vi "LabVIEW.HTTPs_Client.Test_Group.vi"(5 "Chose Server":string, 7 "Command":T1=enum."Test Label", 8 "Fehler (Eingang, kein Fehler)":errorcluster) -> (0 "Fehler (Ausgang)":errorcluster)   [LabVIEW 2026]
uses:
  LabVIEW.Type Definitions/LabVIEW.HTTPs_Client.Test_Group.Command.ctl
  LabVIEW.Type Definitions/LabVIEW.HTTPs_Client.Command.ctl
  <vilib>/JDP Science/JSONtext/String Subset.vi
  <vilib>/JDP Science/JSONtext/support/Strip Quotes and Unescape.vi
  <vilib>/JDP Science/JSONtext/support/Unescape JSON string.vi
  <vilib>/JDP Science/JSONtext/Parsing/Parse Full Path or Item Name.vi
  <vilib>/JDP Science/JSONtext/Offset/Find Item Locations by Path.vi
  <vilib>/JDP Science/JSONtext/JSONtext.lvlib
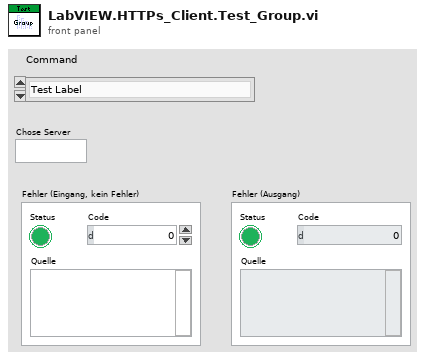
[diagram p1: front panel]
types:
  T1 = typedef "LabVIEW.HTTPs_Client.Test_Group.Command.ctl" = enum16{"No Command", " Test Authentication in the beginning", "Test Label", "Test Seriennummer", "Test Vorgang/Fertigung/Search", "Test User/Role/Permission", "Test MAC addresses", "Test Product/Product properties", "Test Health check", " Test Authentication at the end"}
  T2 = typedef "LabVIEW.HTTPs_Client.Command.ctl" = enum16{"Initialize HTTPS", "Authentication: Creat a token", "Authentication: Get all tokens", "Authentication: Revoke the token", "Label: Creat a label configuration", "Label: Get all configured labels", "Label: Update the label configuration", "Label: Delete the label configuration", "Label: Creat a colour ribbon", "Label: Update the colour ribbon", "Label: Get all colour ribbons", "Label: Delete the colour ribbon", "Label: Creat a label tape", "Label: Update the label tape", "Label: Get all label tapes", "Label: Delete the label tape", "Label: Get all label parameters", "Product: Get all product informations", "Product: Get all reading steps", "Seriennummer: Update the info text", "Seriennummer: Set all step states open", "Seriennummer: Update step states", "Seriennummer: Get data and steps", "Seriennummer: Get all label configurations", "Seriennummer: Create a text report(Prüfbericht)", "Seriennummer: Get the text report(Prüfbericht)", "Seriennummer: Delete the text report(Prüfbericht)", "Seriennummer: Upload a document(txt file)", "Seriennummer: Get the document", "Seriennummer: Get the document thumbnail", "Seriennummer: Delete the document", "Seriennummer: Bulk lookup", "Vorgang: Update the description text", "Vorgang: Migrate serial numbers to a Vorgang", "Vorgang: Migrate serial numbers to a product revision", "Vorgang: Update step states", "Vorgang: Create test reports(Prüfprotokoll)", "Vorgang: Get basic data", "Vorgang: Get serial number data and steps", "Vorgang: Get all serial numbers", "Vorgang: Generate a CSV file", "Vorgang: Generate an XLSX file", "Vorgang: Get a CSV file(Fertigmeldung report)", "Fertigmeldung: Create a Fertigmeldung", "Fertigmeldung: Revert the Fertigmeldung", "User: Get all users", "User: Update an user", "User: Get a single user", "User: Get all user roles", "User: Update a user role", "User: Get a single user role", "User: Get all permissions", "Search: Get Vorgang/Produkt combinations", "Search: Get Vorgang/Produkt/SN combinations", "Search: Get Seriennummern by Vorgang and Produkt", "Search: Lookup Vorgang", "MAC addresses: Get all reserved MAC addresses", "MAC addresses: Get the most recently reserved MAC addresses", "MAC addresses: Get data for a MAC address", "MAC addresses: Reserve MAC addresses for a Seriennummer", "MAC addresses: Mark a reserved MAC address as flashed", "Product: Get possible steps", "Product: Get all products", "Product: Create a new product", "Product: Update a product's data", "Product: Get next product IDs", "Product: Delete a product", "Product properties: Get all product property types", "Search: Find production plan", "Search: Find production plan arrangement", "Health check: Health check", "Deinitialize HTTPs"}
  T3 = enum16{"read csv", "clear csv", "read xlsx", "clear xlsx"}
  T4 = cluster{"Name":string, "URL":string, "Request body":string, "-H":string, "Hearder":string, "Bpdy":string}
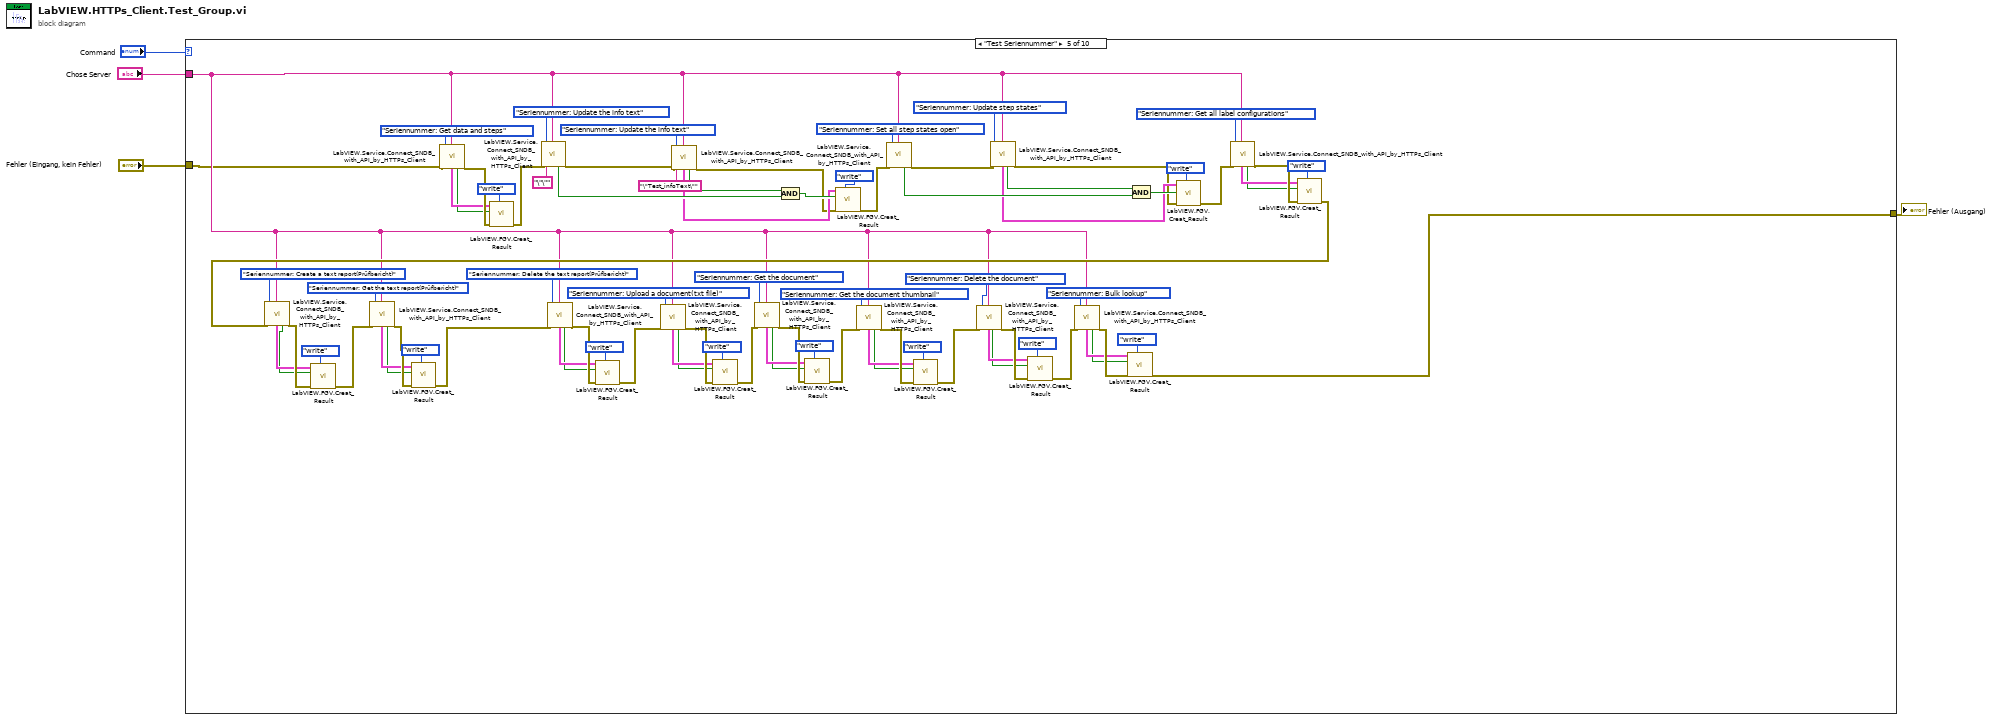
[diagram p0: block diagram]
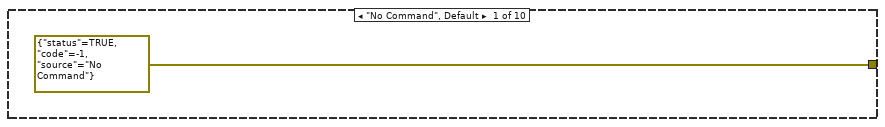
[diagram p2: hidden frame]
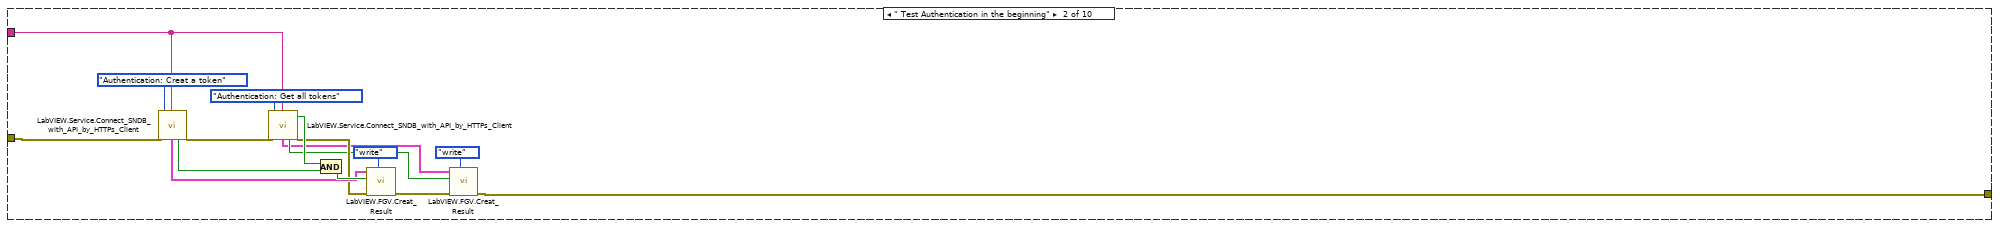
[diagram p3: hidden frame]
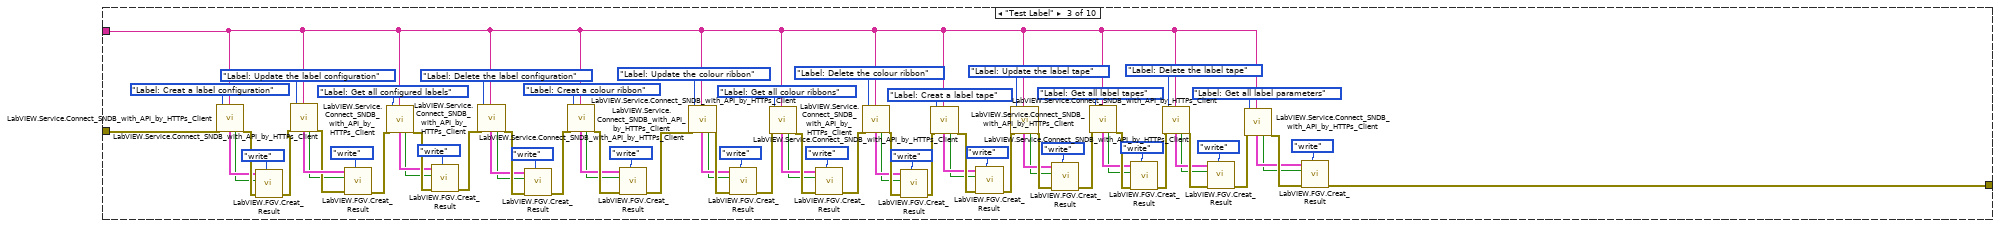
[diagram p4: hidden frame]
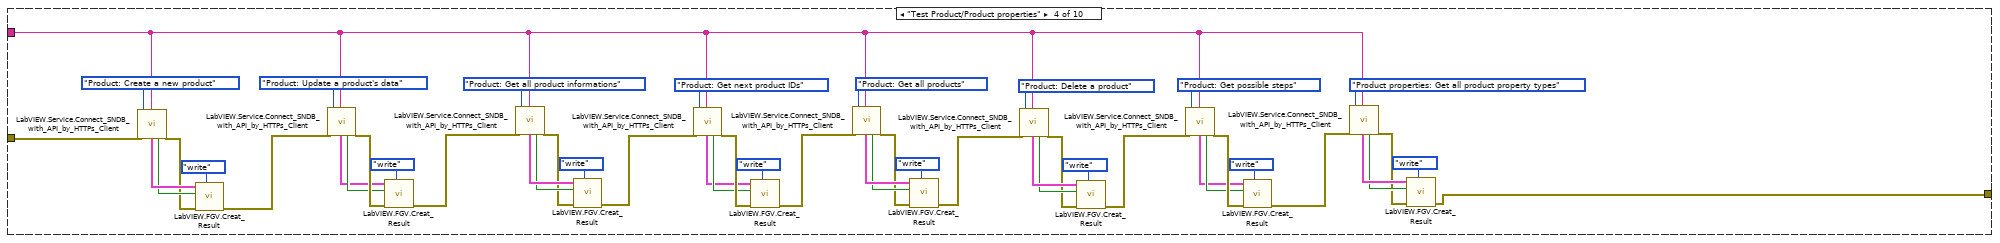
[diagram p5: hidden frame]
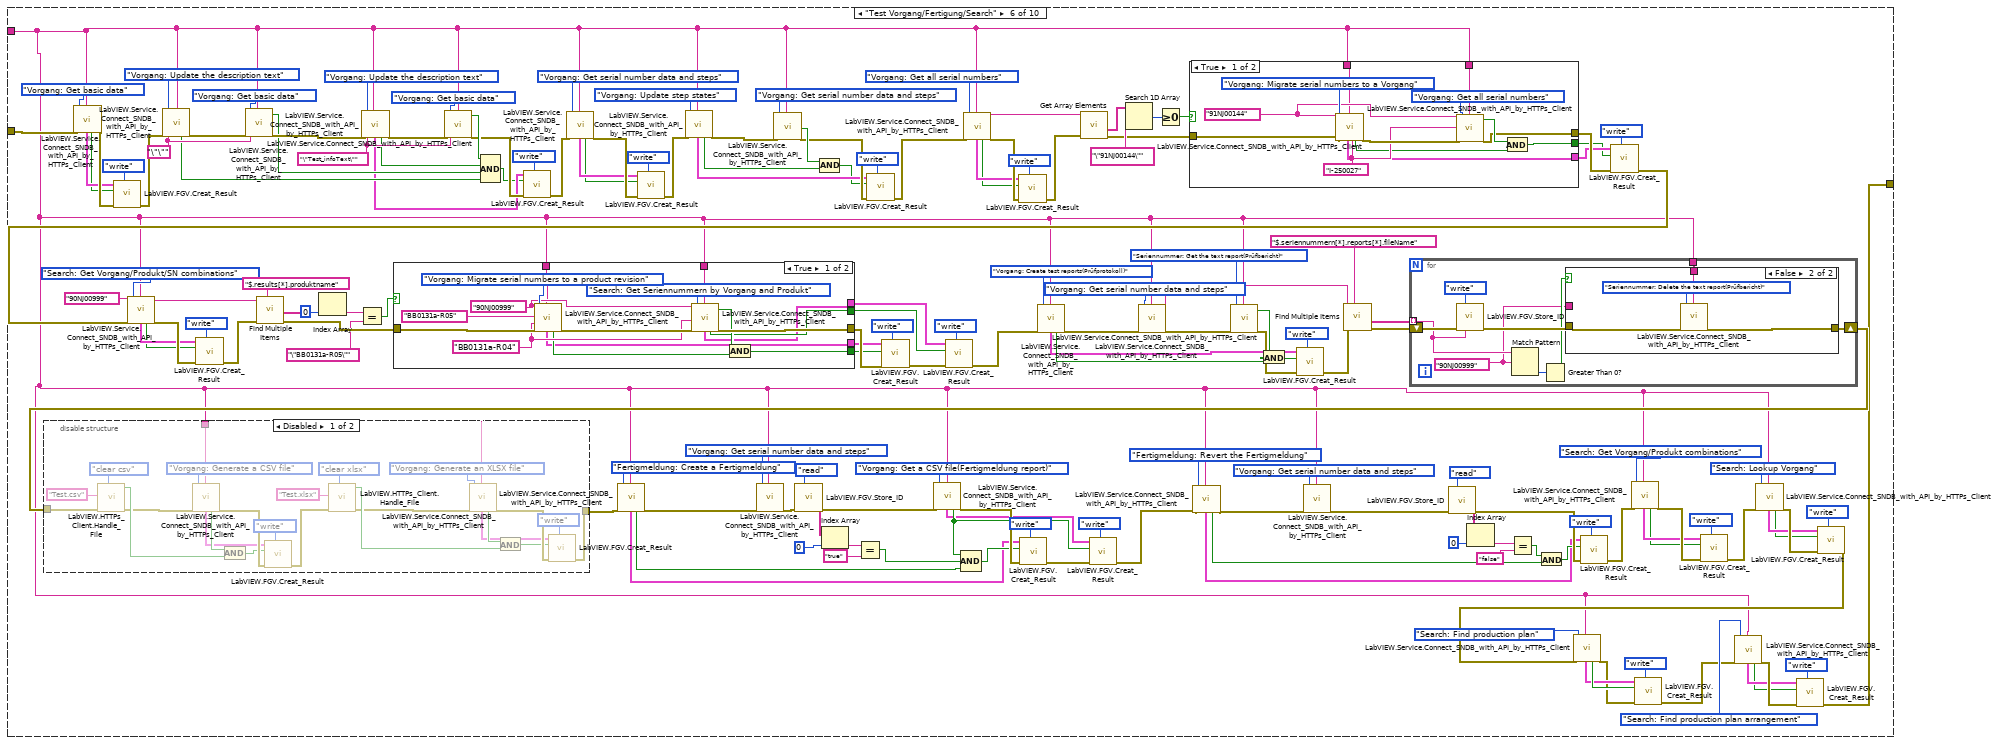
[diagram p6: hidden frame]
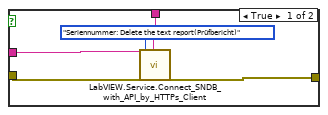
[diagram p8: hidden frame]
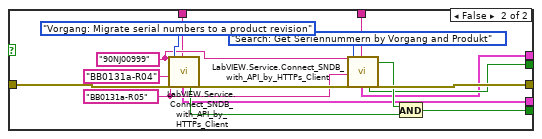
[diagram p9: hidden frame]
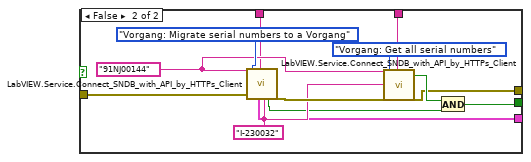
[diagram p10: hidden frame]
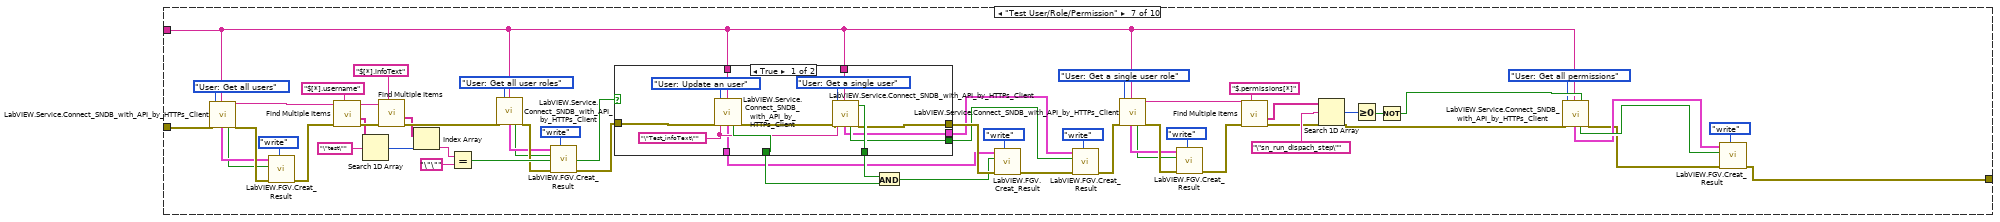
[diagram p11: hidden frame]
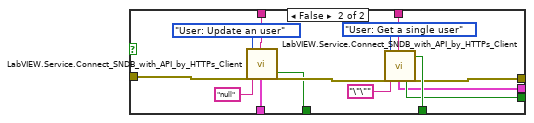
[diagram p12: hidden frame]
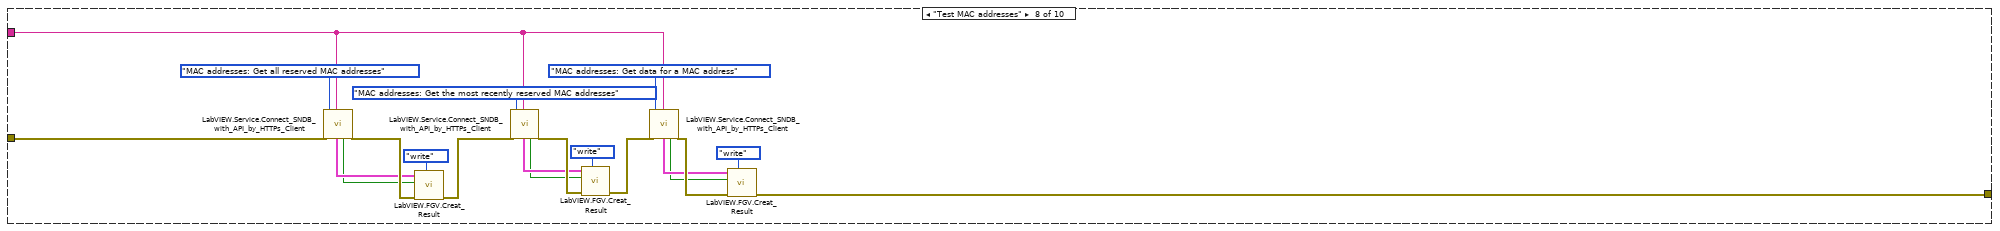
[diagram p13: hidden frame]
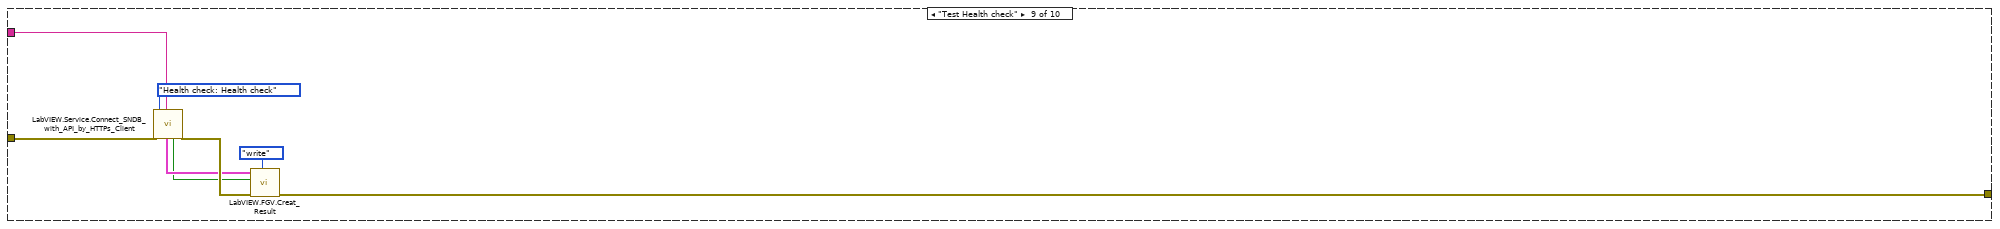
[diagram p14: hidden frame]
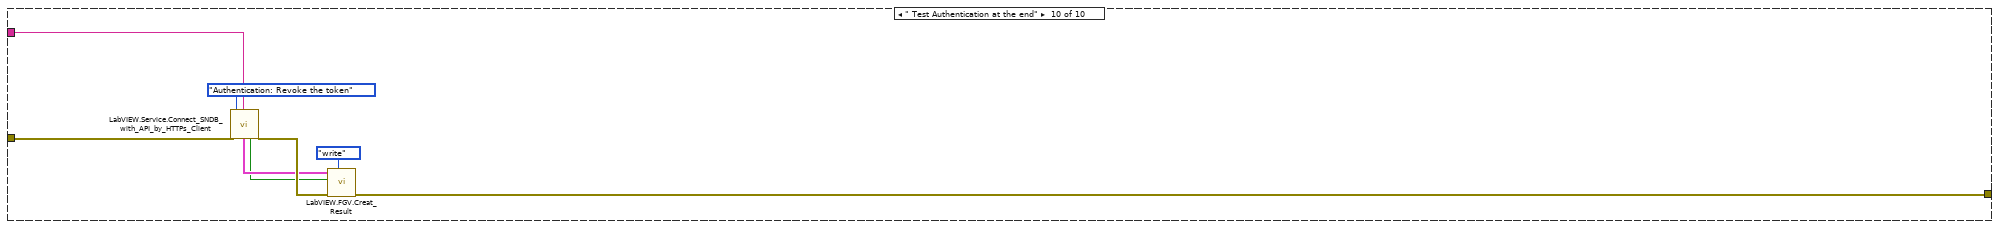
[diagram p15: hidden frame]
diagram:
  n1 = case shown="\"Test Seriennummer\"" "Command" {
    tunnel: "Fehler (Eingang, kein Fehler)" -> [_ w16 w101 w148 w154 w371 w531 w600 w605 w617]
    tunnel: [errorcluster {"status"=TRUE, "code"=-1, "source"="No Command"} ("error out") w7 w25 w102 w156 w237 w503 w587 w604 w615] -> w3
    tunnel: "Chose Server" -> [_ w6 w22 w103 w155 w236 w502 w584 w606 w612]
    frame "No Command", Default {
    }
    frame " Test Authentication in the beginning" {
      n2 = call "LabVIEW.Service.Connect_SNDB_with_API_by_HTTPs_Client.vi"("error in (no error)"=w16, "Command"=LabVIEW.HTTPs_Client.Command."Authentication: Creat a token", "Chose Server"=w6) -> ("Result_Cluster"=w13:T4, "Successful?"=w21:bool, "error out"=w17:errorcluster)  [unwired: 14 in, 8 out]
      n3 = call "LabVIEW.Service.Connect_SNDB_with_API_by_HTTPs_Client.vi"("error in (no error)"=w17, "Command"=LabVIEW.HTTPs_Client.Command."Authentication: Get all tokens", "Chose Server"=w6) -> ("Result_Cluster"=w8:T4, "Successful?"=w9:bool, "Test other steps"=w20:bool, "error out"=w12:errorcluster)  [unwired: 14 in, 7 out]
      n4 = And(x=w20, y=w21) -> (x .and. y?=w14:bool)
      n5 = call "LabVIEW.FGV.Creat_Result.vi"("Command"=enum16{"write", "read", "clear"}."write", "error in (no error)"=w12, "Passed?"=w14, "Result_Cluster"=w13) -> ("error out"=w10:errorcluster)  [unwired: 6 in, 1 out]
      n6 = call "LabVIEW.FGV.Creat_Result.vi"("Command"=enum16{"write", "read", "clear"}."write", "error in (no error)"=w10, "Passed?"=w9, "Result_Cluster"=w8) -> ("error out"=w7:errorcluster)  [unwired: 6 in, 1 out]
    }
    frame "Test Label" {
      n7 = call "LabVIEW.Service.Connect_SNDB_with_API_by_HTTPs_Client.vi"("error in (no error)"=w101, "Command"=LabVIEW.HTTPs_Client.Command."Label: Creat a label configuration", "Chose Server"=w22) -> ("Result_Cluster"=w84:T4, "Successful?"=w83:bool, "error out"=w87:errorcluster)  [unwired: 14 in, 8 out]
      n8 = call "LabVIEW.FGV.Creat_Result.vi"("Command"=enum16{"write", "read", "clear"}."write", "error in (no error)"=w87, "Passed?"=w83, "Result_Cluster"=w84) -> ("error out"=w86:errorcluster)  [unwired: 6 in, 1 out]
      n9 = call "LabVIEW.Service.Connect_SNDB_with_API_by_HTTPs_Client.vi"("error in (no error)"=w86, "Command"=LabVIEW.HTTPs_Client.Command."Label: Update the label configuration", "Chose Server"=w22) -> ("Result_Cluster"=w81:T4, "Successful?"=w78:bool, "error out"=w80:errorcluster)  [unwired: 14 in, 8 out]
      n10 = call "LabVIEW.FGV.Creat_Result.vi"("Command"=enum16{"write", "read", "clear"}."write", "error in (no error)"=w80, "Passed?"=w78, "Result_Cluster"=w81) -> ("error out"=w79:errorcluster)  [unwired: 6 in, 1 out]
      n11 = call "LabVIEW.Service.Connect_SNDB_with_API_by_HTTPs_Client.vi"("error in (no error)"=w79, "Command"=LabVIEW.HTTPs_Client.Command."Label: Get all configured labels", "Chose Server"=w22) -> ("Result_Cluster"=w74:T4, "Successful?"=w73:bool, "error out"=w76:errorcluster)  [unwired: 14 in, 8 out]
      n12 = call "LabVIEW.FGV.Creat_Result.vi"("Command"=enum16{"write", "read", "clear"}."write", "error in (no error)"=w76, "Passed?"=w73, "Result_Cluster"=w74) -> ("error out"=w75:errorcluster)  [unwired: 6 in, 1 out]
      n13 = call "LabVIEW.Service.Connect_SNDB_with_API_by_HTTPs_Client.vi"("error in (no error)"=w75, "Command"=LabVIEW.HTTPs_Client.Command."Label: Delete the label configuration", "Chose Server"=w22) -> ("Result_Cluster"=w69:T4, "Successful?"=w68:bool, "error out"=w71:errorcluster)  [unwired: 14 in, 8 out]
      n14 = call "LabVIEW.FGV.Creat_Result.vi"("Command"=enum16{"write", "read", "clear"}."write", "error in (no error)"=w71, "Passed?"=w68, "Result_Cluster"=w69) -> ("error out"=w70:errorcluster)  [unwired: 6 in, 1 out]
      n15 = call "LabVIEW.Service.Connect_SNDB_with_API_by_HTTPs_Client.vi"("error in (no error)"=w70, "Command"=LabVIEW.HTTPs_Client.Command."Label: Creat a colour ribbon", "Chose Server"=w22) -> ("Result_Cluster"=w64:T4, "Successful?"=w63:bool, "error out"=w66:errorcluster)  [unwired: 14 in, 8 out]
      n16 = call "LabVIEW.FGV.Creat_Result.vi"("Command"=enum16{"write", "read", "clear"}."write", "error in (no error)"=w66, "Passed?"=w63, "Result_Cluster"=w64) -> ("error out"=w65:errorcluster)  [unwired: 6 in, 1 out]
      n17 = call "LabVIEW.Service.Connect_SNDB_with_API_by_HTTPs_Client.vi"("error in (no error)"=w65, "Command"=LabVIEW.HTTPs_Client.Command."Label: Update the colour ribbon", "Chose Server"=w22) -> ("Result_Cluster"=w60:T4, "Successful?"=w59:bool, "error out"=w61:errorcluster)  [unwired: 14 in, 8 out]
      n18 = call "LabVIEW.FGV.Creat_Result.vi"("Command"=enum16{"write", "read", "clear"}."write", "error in (no error)"=w61, "Passed?"=w59, "Result_Cluster"=w60) -> ("error out"=w58:errorcluster)  [unwired: 6 in, 1 out]
      n19 = call "LabVIEW.Service.Connect_SNDB_with_API_by_HTTPs_Client.vi"("error in (no error)"=w58, "Command"=LabVIEW.HTTPs_Client.Command."Label: Get all colour ribbons", "Chose Server"=w22) -> ("Result_Cluster"=w54:T4, "Successful?"=w53:bool, "error out"=w56:errorcluster)  [unwired: 14 in, 8 out]
      n20 = call "LabVIEW.FGV.Creat_Result.vi"("Command"=enum16{"write", "read", "clear"}."write", "error in (no error)"=w56, "Passed?"=w53, "Result_Cluster"=w54) -> ("error out"=w55:errorcluster)  [unwired: 6 in, 1 out]
      n21 = call "LabVIEW.Service.Connect_SNDB_with_API_by_HTTPs_Client.vi"("error in (no error)"=w55, "Command"=LabVIEW.HTTPs_Client.Command."Label: Delete the colour ribbon", "Chose Server"=w22) -> ("Result_Cluster"=w49:T4, "Successful?"=w48:bool, "error out"=w51:errorcluster)  [unwired: 14 in, 8 out]
      n22 = call "LabVIEW.FGV.Creat_Result.vi"("Command"=enum16{"write", "read", "clear"}."write", "error in (no error)"=w51, "Passed?"=w48, "Result_Cluster"=w49) -> ("error out"=w50:errorcluster)  [unwired: 6 in, 1 out]
      n23 = call "LabVIEW.Service.Connect_SNDB_with_API_by_HTTPs_Client.vi"("error in (no error)"=w50, "Command"=LabVIEW.HTTPs_Client.Command."Label: Creat a label tape", "Chose Server"=w22) -> ("Result_Cluster"=w44:T4, "Successful?"=w43:bool, "error out"=w46:errorcluster)  [unwired: 14 in, 8 out]
      n24 = call "LabVIEW.FGV.Creat_Result.vi"("Command"=enum16{"write", "read", "clear"}."write", "error in (no error)"=w46, "Passed?"=w43, "Result_Cluster"=w44) -> ("error out"=w45:errorcluster)  [unwired: 6 in, 1 out]
      n25 = call "LabVIEW.Service.Connect_SNDB_with_API_by_HTTPs_Client.vi"("error in (no error)"=w45, "Command"=LabVIEW.HTTPs_Client.Command."Label: Update the label tape", "Chose Server"=w22) -> ("Result_Cluster"=w39:T4, "Successful?"=w38:bool, "error out"=w41:errorcluster)  [unwired: 14 in, 8 out]
      n26 = call "LabVIEW.FGV.Creat_Result.vi"("Command"=enum16{"write", "read", "clear"}."write", "error in (no error)"=w41, "Passed?"=w38, "Result_Cluster"=w39) -> ("error out"=w40:errorcluster)  [unwired: 6 in, 1 out]
      n27 = call "LabVIEW.Service.Connect_SNDB_with_API_by_HTTPs_Client.vi"("error in (no error)"=w40, "Command"=LabVIEW.HTTPs_Client.Command."Label: Get all label tapes", "Chose Server"=w22) -> ("Result_Cluster"=w34:T4, "Successful?"=w33:bool, "error out"=w36:errorcluster)  [unwired: 14 in, 8 out]
      n28 = call "LabVIEW.FGV.Creat_Result.vi"("Command"=enum16{"write", "read", "clear"}."write", "error in (no error)"=w36, "Passed?"=w33, "Result_Cluster"=w34) -> ("error out"=w35:errorcluster)  [unwired: 6 in, 1 out]
      n29 = call "LabVIEW.Service.Connect_SNDB_with_API_by_HTTPs_Client.vi"("error in (no error)"=w35, "Command"=LabVIEW.HTTPs_Client.Command."Label: Delete the label tape", "Chose Server"=w22) -> ("Result_Cluster"=w30:T4, "Successful?"=w29:bool, "error out"=w31:errorcluster)  [unwired: 14 in, 8 out]
      n30 = call "LabVIEW.FGV.Creat_Result.vi"("Command"=enum16{"write", "read", "clear"}."write", "error in (no error)"=w31, "Passed?"=w29, "Result_Cluster"=w30) -> ("error out"=w28:errorcluster)  [unwired: 6 in, 1 out]
      n31 = call "LabVIEW.Service.Connect_SNDB_with_API_by_HTTPs_Client.vi"("error in (no error)"=w28, "Command"=LabVIEW.HTTPs_Client.Command."Label: Get all label parameters", "Chose Server"=w22) -> ("Result_Cluster"=w24:T4, "Successful?"=w23:bool, "error out"=w26:errorcluster)  [unwired: 14 in, 8 out]
      n32 = call "LabVIEW.FGV.Creat_Result.vi"("Command"=enum16{"write", "read", "clear"}."write", "error in (no error)"=w26, "Passed?"=w23, "Result_Cluster"=w24) -> ("error out"=w25:errorcluster)  [unwired: 6 in, 1 out]
    }
    frame "Test Product/Product properties" {
      n33 = call "LabVIEW.Service.Connect_SNDB_with_API_by_HTTPs_Client.vi"("error in (no error)"=w148, "Command"=LabVIEW.HTTPs_Client.Command."Product: Create a new product", "Chose Server"=w103) -> ("Result_Cluster"=w150:T4, "Successful?"=w149:bool, "error out"=w146:errorcluster)  [unwired: 14 in, 8 out]
      n34 = call "LabVIEW.FGV.Creat_Result.vi"("Command"=enum16{"write", "read", "clear"}."write", "error in (no error)"=w146, "Passed?"=w149, "Result_Cluster"=w150) -> ("error out"=w140:errorcluster)  [unwired: 6 in, 1 out]
      n35 = call "LabVIEW.Service.Connect_SNDB_with_API_by_HTTPs_Client.vi"("error in (no error)"=w140, "Command"=LabVIEW.HTTPs_Client.Command."Product: Update a product's data", "Chose Server"=w103) -> ("Result_Cluster"=w142:T4, "Successful?"=w143:bool, "error out"=w145:errorcluster)  [unwired: 14 in, 8 out]
      n36 = call "LabVIEW.FGV.Creat_Result.vi"("Command"=enum16{"write", "read", "clear"}."write", "error in (no error)"=w145, "Passed?"=w143, "Result_Cluster"=w142) -> ("error out"=w134:errorcluster)  [unwired: 6 in, 1 out]
      n37 = call "LabVIEW.Service.Connect_SNDB_with_API_by_HTTPs_Client.vi"("error in (no error)"=w134, "Command"=LabVIEW.HTTPs_Client.Command."Product: Get all product informations", "Chose Server"=w103) -> ("Result_Cluster"=w138:T4, "Successful?"=w137:bool, "error out"=w135:errorcluster)  [unwired: 14 in, 8 out]
      n38 = call "LabVIEW.FGV.Creat_Result.vi"("Command"=enum16{"write", "read", "clear"}."write", "error in (no error)"=w135, "Passed?"=w137, "Result_Cluster"=w138) -> ("error out"=w128:errorcluster)  [unwired: 6 in, 1 out]
      n39 = call "LabVIEW.Service.Connect_SNDB_with_API_by_HTTPs_Client.vi"("error in (no error)"=w128, "Command"=LabVIEW.HTTPs_Client.Command."Product: Get next product IDs", "Chose Server"=w103) -> ("Result_Cluster"=w130:T4, "Successful?"=w131:bool, "error out"=w133:errorcluster)  [unwired: 14 in, 8 out]
      n40 = call "LabVIEW.FGV.Creat_Result.vi"("Command"=enum16{"write", "read", "clear"}."write", "error in (no error)"=w133, "Passed?"=w131, "Result_Cluster"=w130) -> ("error out"=w122:errorcluster)  [unwired: 6 in, 1 out]
      n41 = call "LabVIEW.Service.Connect_SNDB_with_API_by_HTTPs_Client.vi"("error in (no error)"=w122, "Command"=LabVIEW.HTTPs_Client.Command."Product: Get all products", "Chose Server"=w103) -> ("Result_Cluster"=w126:T4, "Successful?"=w125:bool, "error out"=w123:errorcluster)  [unwired: 14 in, 8 out]
      n42 = call "LabVIEW.FGV.Creat_Result.vi"("Command"=enum16{"write", "read", "clear"}."write", "error in (no error)"=w123, "Passed?"=w125, "Result_Cluster"=w126) -> ("error out"=w111:errorcluster)  [unwired: 6 in, 1 out]
      n43 = call "LabVIEW.Service.Connect_SNDB_with_API_by_HTTPs_Client.vi"("error in (no error)"=w111, "Command"=LabVIEW.HTTPs_Client.Command."Product: Delete a product", "Chose Server"=w103) -> ("Result_Cluster"=w115:T4, "Successful?"=w114:bool, "error out"=w112:errorcluster)  [unwired: 14 in, 8 out]
      n44 = call "LabVIEW.FGV.Creat_Result.vi"("Command"=enum16{"write", "read", "clear"}."write", "error in (no error)"=w112, "Passed?"=w114, "Result_Cluster"=w115) -> ("error out"=w105:errorcluster)  [unwired: 6 in, 1 out]
      n45 = call "LabVIEW.Service.Connect_SNDB_with_API_by_HTTPs_Client.vi"("error in (no error)"=w105, "Command"=LabVIEW.HTTPs_Client.Command."Product: Get possible steps", "Chose Server"=w103) -> ("Result_Cluster"=w118:T4, "Successful?"=w119:bool, "error out"=w121:errorcluster)  [unwired: 14 in, 8 out]
      n46 = call "LabVIEW.FGV.Creat_Result.vi"("Command"=enum16{"write", "read", "clear"}."write", "error in (no error)"=w121, "Passed?"=w119, "Result_Cluster"=w118) -> ("error out"=w104:errorcluster)  [unwired: 6 in, 1 out]
      n47 = call "LabVIEW.Service.Connect_SNDB_with_API_by_HTTPs_Client.vi"("error in (no error)"=w104, "Command"=LabVIEW.HTTPs_Client.Command."Product properties: Get all product property types", "Chose Server"=w103) -> ("Result_Cluster"=w109:T4, "Successful?"=w108:bool, "error out"=w106:errorcluster)  [unwired: 14 in, 8 out]
      n48 = call "LabVIEW.FGV.Creat_Result.vi"("Command"=enum16{"write", "read", "clear"}."write", "error in (no error)"=w106, "Passed?"=w108, "Result_Cluster"=w109) -> ("error out"=w102:errorcluster)  [unwired: 6 in, 1 out]
    }
    frame "Test Seriennummer" {
      n49 = call "LabVIEW.Service.Connect_SNDB_with_API_by_HTTPs_Client.vi"("error in (no error)"=w154, "Command"=LabVIEW.HTTPs_Client.Command."Seriennummer: Get data and steps", "Chose Server"=w155) -> ("Result_Cluster"=w218:T4, "Successful?"=w217:bool, "error out"=w220:errorcluster)  [unwired: 14 in, 8 out]
      n50 = call "LabVIEW.FGV.Creat_Result.vi"("Command"=enum16{"write", "read", "clear"}."write", "error in (no error)"=w220, "Passed?"=w217, "Result_Cluster"=w218) -> ("error out"=w219:errorcluster)  [unwired: 6 in, 1 out]
      n51 = call "LabVIEW.Service.Connect_SNDB_with_API_by_HTTPs_Client.vi"("error in (no error)"=w219, "Command"=LabVIEW.HTTPs_Client.Command."Seriennummer: Update the info text", "Info text"="\"\"" ("SN: Info text"), "Chose Server"=w155) -> ("Successful?"=w229:bool, "error out"=w232:errorcluster)  [unwired: 13 in, 9 out]
      n52 = call "LabVIEW.Service.Connect_SNDB_with_API_by_HTTPs_Client.vi"("error in (no error)"=w232, "Command"=LabVIEW.HTTPs_Client.Command."Seriennummer: Update the info text", "Info text"="\"Test_infoText\"" ("SN: Info text"), "Chose Server"=w155) -> ("Result_Cluster"=w213:T4, "Successful?"=w230:bool, "error out"=w153:errorcluster)  [unwired: 13 in, 8 out]
      n53 = Compound Arithmetic op=AND ("Mehrfacharithmetik")(w230, w229) -> (w214:bool)
      n54 = call "LabVIEW.FGV.Creat_Result.vi"("Command"=enum16{"write", "read", "clear"}."write", "error in (no error)"=w153, "Passed?"=w214, "Result_Cluster"=w213) -> ("error out"=w215:errorcluster)  [unwired: 6 in, 1 out]
      n55 = call "LabVIEW.Service.Connect_SNDB_with_API_by_HTTPs_Client.vi"("error in (no error)"=w215, "Command"=LabVIEW.HTTPs_Client.Command."Seriennummer: Set all step states open", "Chose Server"=w155) -> ("Successful?"=w224:bool, "error out"=w226:errorcluster)  [unwired: 14 in, 9 out]
      n56 = call "LabVIEW.Service.Connect_SNDB_with_API_by_HTTPs_Client.vi"("error in (no error)"=w226, "Command"=LabVIEW.HTTPs_Client.Command."Seriennummer: Update step states", "Chose Server"=w155) -> ("Result_Cluster"=w209:T4, "Successful?"=w225:bool, "error out"=w152:errorcluster)  [unwired: 14 in, 8 out]
      n57 = Compound Arithmetic op=AND ("Mehrfacharithmetik")(w225, w224) -> (w210:bool)
      n58 = call "LabVIEW.FGV.Creat_Result.vi"("Command"=enum16{"write", "read", "clear"}."write", "error in (no error)"=w152, "Passed?"=w210, "Result_Cluster"=w209) -> ("error out"=w211:errorcluster)  [unwired: 6 in, 1 out]
      n59 = call "LabVIEW.Service.Connect_SNDB_with_API_by_HTTPs_Client.vi"("error in (no error)"=w211, "Command"=LabVIEW.HTTPs_Client.Command."Seriennummer: Get all label configurations", "Chose Server"=w155) -> ("Result_Cluster"=w206:T4, "Successful?"=w205:bool, "error out"=w207:errorcluster)  [unwired: 14 in, 8 out]
      n60 = call "LabVIEW.FGV.Creat_Result.vi"("Command"=enum16{"write", "read", "clear"}."write", "error in (no error)"=w207, "Passed?"=w205, "Result_Cluster"=w206) -> ("error out"=w196:errorcluster)  [unwired: 6 in, 1 out]
      n61 = call "LabVIEW.Service.Connect_SNDB_with_API_by_HTTPs_Client.vi"("error in (no error)"=w196, "Command"=LabVIEW.HTTPs_Client.Command."Seriennummer: Create a text report(Prüfbericht)", "Chose Server"=w155) -> ("Result_Cluster"=w191:T4, "Successful?"=w190:bool, "error out"=w193:errorcluster)  [unwired: 14 in, 8 out]
      n62 = call "LabVIEW.FGV.Creat_Result.vi"("Command"=enum16{"write", "read", "clear"}."write", "error in (no error)"=w193, "Passed?"=w190, "Result_Cluster"=w191) -> ("error out"=w192:errorcluster)  [unwired: 6 in, 1 out]
      n63 = call "LabVIEW.Service.Connect_SNDB_with_API_by_HTTPs_Client.vi"("error in (no error)"=w192, "Command"=LabVIEW.HTTPs_Client.Command."Seriennummer: Get the text report(Prüfbericht)", "Chose Server"=w155) -> ("Result_Cluster"=w187:T4, "Successful?"=w186:bool, "error out"=w189:errorcluster)  [unwired: 14 in, 8 out]
      n64 = call "LabVIEW.FGV.Creat_Result.vi"("Command"=enum16{"write", "read", "clear"}."write", "error in (no error)"=w189, "Passed?"=w186, "Result_Cluster"=w187) -> ("error out"=w188:errorcluster)  [unwired: 6 in, 1 out]
      n65 = call "LabVIEW.Service.Connect_SNDB_with_API_by_HTTPs_Client.vi"("error in (no error)"=w188, "Command"=LabVIEW.HTTPs_Client.Command."Seriennummer: Delete the text report(Prüfbericht)", "Chose Server"=w155) -> ("Result_Cluster"=w182:T4, "Successful?"=w181:bool, "error out"=w184:errorcluster)  [unwired: 14 in, 8 out]
      n66 = call "LabVIEW.FGV.Creat_Result.vi"("Command"=enum16{"write", "read", "clear"}."write", "error in (no error)"=w184, "Passed?"=w181, "Result_Cluster"=w182) -> ("error out"=w183:errorcluster)  [unwired: 6 in, 1 out]
      n67 = call "LabVIEW.Service.Connect_SNDB_with_API_by_HTTPs_Client.vi"("error in (no error)"=w183, "Command"=LabVIEW.HTTPs_Client.Command."Seriennummer: Upload a document(txt file)", "Chose Server"=w155) -> ("Result_Cluster"=w177:T4, "Successful?"=w176:bool, "error out"=w179:errorcluster)  [unwired: 14 in, 8 out]
      n68 = call "LabVIEW.FGV.Creat_Result.vi"("Command"=enum16{"write", "read", "clear"}."write", "error in (no error)"=w179, "Passed?"=w176, "Result_Cluster"=w177) -> ("error out"=w178:errorcluster)  [unwired: 6 in, 1 out]
      n69 = call "LabVIEW.Service.Connect_SNDB_with_API_by_HTTPs_Client.vi"("error in (no error)"=w178, "Command"=LabVIEW.HTTPs_Client.Command."Seriennummer: Get the document", "Chose Server"=w155) -> ("Result_Cluster"=w172:T4, "Successful?"=w171:bool, "error out"=w174:errorcluster)  [unwired: 14 in, 8 out]
      n70 = call "LabVIEW.FGV.Creat_Result.vi"("Command"=enum16{"write", "read", "clear"}."write", "error in (no error)"=w174, "Passed?"=w171, "Result_Cluster"=w172) -> ("error out"=w173:errorcluster)  [unwired: 6 in, 1 out]
      n71 = call "LabVIEW.Service.Connect_SNDB_with_API_by_HTTPs_Client.vi"("error in (no error)"=w173, "Command"=LabVIEW.HTTPs_Client.Command."Seriennummer: Get the document thumbnail", "Chose Server"=w155) -> ("Result_Cluster"=w167:T4, "Successful?"=w166:bool, "error out"=w169:errorcluster)  [unwired: 14 in, 8 out]
      n72 = call "LabVIEW.FGV.Creat_Result.vi"("Command"=enum16{"write", "read", "clear"}."write", "error in (no error)"=w169, "Passed?"=w166, "Result_Cluster"=w167) -> ("error out"=w168:errorcluster)  [unwired: 6 in, 1 out]
      n73 = call "LabVIEW.Service.Connect_SNDB_with_API_by_HTTPs_Client.vi"("error in (no error)"=w168, "Command"=LabVIEW.HTTPs_Client.Command."Seriennummer: Delete the document", "Chose Server"=w155) -> ("Result_Cluster"=w162:T4, "Successful?"=w161:bool, "error out"=w164:errorcluster)  [unwired: 14 in, 8 out]
      n74 = call "LabVIEW.FGV.Creat_Result.vi"("Command"=enum16{"write", "read", "clear"}."write", "error in (no error)"=w164, "Passed?"=w161, "Result_Cluster"=w162) -> ("error out"=w163:errorcluster)  [unwired: 6 in, 1 out]
      n75 = call "LabVIEW.Service.Connect_SNDB_with_API_by_HTTPs_Client.vi"("error in (no error)"=w163, "Command"=LabVIEW.HTTPs_Client.Command."Seriennummer: Bulk lookup", "Chose Server"=w155) -> ("Result_Cluster"=w158:T4, "Successful?"=w157:bool, "error out"=w159:errorcluster)  [unwired: 14 in, 8 out]
      n76 = call "LabVIEW.FGV.Creat_Result.vi"("Command"=enum16{"write", "read", "clear"}."write", "error in (no error)"=w159, "Passed?"=w157, "Result_Cluster"=w158) -> ("error out"=w156:errorcluster)  [unwired: 6 in, 1 out]
    }
    frame "Test Vorgang/Fertigung/Search" {
      w391 = "\"Test_infoText\"" ("Info text")
      w394 = "\"\"" ("Info text")
      n77 = call "LabVIEW.Service.Connect_SNDB_with_API_by_HTTPs_Client.vi"("error in (no error)"=w371, "Command"=LabVIEW.HTTPs_Client.Command."Vorgang: Get basic data", "Chose Server"=w236) -> ("Result_Cluster"=w367:T4, "Successful?"=w366:bool, "error out"=w369:errorcluster)  [unwired: 14 in, 8 out]
      n78 = call "LabVIEW.FGV.Creat_Result.vi"("Command"=enum16{"write", "read", "clear"}."write", "error in (no error)"=w369, "Passed?"=w366, "Result_Cluster"=w367) -> ("error out"=w368:errorcluster)  [unwired: 6 in, 1 out]
      n79 = call "LabVIEW.Service.Connect_SNDB_with_API_by_HTTPs_Client.vi"("error in (no error)"=w368, "Command"=LabVIEW.HTTPs_Client.Command."Vorgang: Update the description text", "Info text"=w394, "Chose Server"=w236) -> ("Successful?"=w385:bool, "error out"=w395:errorcluster)  [unwired: 13 in, 9 out]
      n80 = call "LabVIEW.Service.Connect_SNDB_with_API_by_HTTPs_Client.vi"("error in (no error)"=w395, "Command"=LabVIEW.HTTPs_Client.Command."Vorgang: Get basic data", "Info text"=w394, "Chose Server"=w236) -> ("Test other steps"=w386:bool, "error out"=w389:errorcluster)  [unwired: 13 in, 9 out]
      n81 = call "LabVIEW.Service.Connect_SNDB_with_API_by_HTTPs_Client.vi"("error in (no error)"=w389, "Command"=LabVIEW.HTTPs_Client.Command."Vorgang: Update the description text", "Info text"=w391, "Chose Server"=w236) -> ("Result_Cluster"=w362:T4, "Successful?"=w387:bool, "error out"=w393:errorcluster)  [unwired: 13 in, 8 out]
      n82 = call "LabVIEW.Service.Connect_SNDB_with_API_by_HTTPs_Client.vi"("error in (no error)"=w393, "Command"=LabVIEW.HTTPs_Client.Command."Vorgang: Get basic data", "Info text"=w391, "Chose Server"=w236) -> ("Test other steps"=w388:bool, "error out"=w364:errorcluster)  [unwired: 13 in, 9 out]
      n83 = Compound Arithmetic op=AND ("Mehrfacharithmetik")(w388, w387, w386, w385) -> (w361:bool)
      n84 = call "LabVIEW.FGV.Creat_Result.vi"("Command"=enum16{"write", "read", "clear"}."write", "error in (no error)"=w364, "Passed?"=w361, "Result_Cluster"=w362) -> ("error out"=w363:errorcluster)  [unwired: 6 in, 1 out]
      n85 = call "LabVIEW.Service.Connect_SNDB_with_API_by_HTTPs_Client.vi"("error in (no error)"=w363, "Command"=LabVIEW.HTTPs_Client.Command."Vorgang: Get serial number data and steps", "Chose Server"=w236) -> ("Result_Cluster"=w357:T4, "Successful?"=w356:bool, "error out"=w359:errorcluster)  [unwired: 14 in, 8 out]
      n86 = call "LabVIEW.FGV.Creat_Result.vi"("Command"=enum16{"write", "read", "clear"}."write", "error in (no error)"=w359, "Passed?"=w356, "Result_Cluster"=w357) -> ("error out"=w358:errorcluster)  [unwired: 6 in, 1 out]
      n87 = call "LabVIEW.Service.Connect_SNDB_with_API_by_HTTPs_Client.vi"("error in (no error)"=w358, "Command"=LabVIEW.HTTPs_Client.Command."Vorgang: Update step states", "Chose Server"=w236) -> ("Result_Cluster"=w352:T4, "Successful?"=w380:bool, "error out"=w382:errorcluster)  [unwired: 14 in, 8 out]
      n88 = call "LabVIEW.Service.Connect_SNDB_with_API_by_HTTPs_Client.vi"("error in (no error)"=w382, "Command"=LabVIEW.HTTPs_Client.Command."Vorgang: Get serial number data and steps", "Chose Server"=w236) -> ("Test other steps 2"=w379:bool, "error out"=w354:errorcluster)  [unwired: 14 in, 9 out]
      n89 = Compound Arithmetic op=AND ("Mehrfacharithmetik")(w379, w380) -> (w351:bool)
      n90 = call "LabVIEW.FGV.Creat_Result.vi"("Command"=enum16{"write", "read", "clear"}."write", "error in (no error)"=w354, "Passed?"=w351, "Result_Cluster"=w352) -> ("error out"=w353:errorcluster)  [unwired: 6 in, 1 out]
      n91 = call "LabVIEW.Service.Connect_SNDB_with_API_by_HTTPs_Client.vi"("error in (no error)"=w353, "Command"=LabVIEW.HTTPs_Client.Command."Vorgang: Get all serial numbers", "Chose Server"=w236) -> ("Result_Cluster"=w347:T4, "Successful?"=w346:bool, "Body"=w375:string, "error out"=w349:errorcluster)  [unwired: 14 in, 7 out]
      n92 = call "LabVIEW.FGV.Creat_Result.vi"("Command"=enum16{"write", "read", "clear"}."write", "error in (no error)"=w349, "Passed?"=w346, "Result_Cluster"=w347) -> ("error out"=w348:errorcluster)  [unwired: 6 in, 1 out]
      n93 = call <vilib>:"Get Array Elements.vi"("error in (no error)"=w348, "JSON"=w375) -> ("error out"=w372:errorcluster, "<JSON>"=w377:string[])  [unwired: 7 in, 1 out]
      n94 = Search 1D Array(1D array=w377, element="\"91NJ00144\"" ("Info text")) -> (index of element=w376:i32)  [unwired: 1 in]
      n95 = Greater Or Equal To 0?(x=w376) -> (x >= 0?=w373:bool)
      n96 = case shown="True" w373 {
        tunnel: w372 -> [w480 w493]
        tunnel: [w478 w491] -> w344
        tunnel: [w477 w489] -> w343
        tunnel: [w476 w490] -> w342
        tunnel: w236 -> [w475 w488]
        tunnel: w236 -> [w474 w487]
        frame True {
          w481 = "91NJ00144" ("Migrated Vorgang")
          w483 = "I-250027" ("Migrated Vorgang")
          n97 = call "LabVIEW.Service.Connect_SNDB_with_API_by_HTTPs_Client.vi"("SN"=w481, "error in (no error)"=w480, "Command"=LabVIEW.HTTPs_Client.Command."Vorgang: Migrate serial numbers to a Vorgang", "Chose Server"=w475, "Migrated Vorgang"=w483) -> ("Result_Cluster"=w477:T4, "Successful?"=w482:bool, "error out"=w484:errorcluster)  [unwired: 12 in, 8 out]
          n98 = call "LabVIEW.Service.Connect_SNDB_with_API_by_HTTPs_Client.vi"("SN"=w481, "VrN"=w483, "error in (no error)"=w484, "Command"=LabVIEW.HTTPs_Client.Command."Vorgang: Get all serial numbers", "Chose Server"=w474) -> ("Test other steps"=w479:bool, "error out"=w478:errorcluster)  [unwired: 12 in, 9 out]
          n99 = And(x=w479, y=w482) -> (x .and. y?=w476:bool)
        }
        frame False {
          w494 = "91NJ00144" ("Migrated Vorgang")
          w496 = "I-230032" ("Migrated Vorgang")
          n100 = call "LabVIEW.Service.Connect_SNDB_with_API_by_HTTPs_Client.vi"("SN"=w494, "error in (no error)"=w493, "Command"=LabVIEW.HTTPs_Client.Command."Vorgang: Migrate serial numbers to a Vorgang", "Chose Server"=w488, "Migrated Vorgang"=w496) -> ("Result_Cluster"=w489:T4, "Successful?"=w495:bool, "error out"=w497:errorcluster)  [unwired: 12 in, 8 out]
          n101 = call "LabVIEW.Service.Connect_SNDB_with_API_by_HTTPs_Client.vi"("SN"=w494, "VrN"=w496, "error in (no error)"=w497, "Command"=LabVIEW.HTTPs_Client.Command."Vorgang: Get all serial numbers", "Chose Server"=w487) -> ("Test other steps"=w492:bool, "error out"=w491:errorcluster)  [unwired: 12 in, 9 out]
          n102 = And(x=w492, y=w495) -> (x .and. y?=w490:bool)
        }
      }
      n103 = call "LabVIEW.FGV.Creat_Result.vi"("Command"=enum16{"write", "read", "clear"}."write", "error in (no error)"=w344, "Passed?"=w342, "Result_Cluster"=w343) -> ("error out"=w323:errorcluster)  [unwired: 6 in, 1 out]
      n104 = call "LabVIEW.Service.Connect_SNDB_with_API_by_HTTPs_Client.vi"("SN"="90NJ00999", "error in (no error)"=w323, "Command"=LabVIEW.HTTPs_Client.Command."Search: Get Vorgang/Produkt/SN combinations", "Chose Server"=w236) -> ("Result_Cluster"=w319:T4, "Successful?"=w318:bool, "Body"=w341:string, "error out"=w321:errorcluster)  [unwired: 13 in, 7 out]
      n105 = call "LabVIEW.FGV.Creat_Result.vi"("Command"=enum16{"write", "read", "clear"}."write", "error in (no error)"=w321, "Passed?"=w318, "Result_Cluster"=w319) -> ("error out"=w320:errorcluster)  [unwired: 6 in, 1 out]
      n106 = call <vilib>:"Find Multiple Items.vi"("$Path or Item Name"="$.results[*].produktname", "error in (no error)"=w320, "JSON"=w341) -> ("error out"=w332:errorcluster, "<JSON>"=w327:string[])  [unwired: 5 in, 2 out]
      n107 = Index Array(array=w327, index=0 ("Index")) -> (element=w329:string)
      n108 = Equal?(x=w329, y="\"BB0131a-R05\"") -> (x = y?=w331:bool)
      n109 = case shown="True" w331 {
        tunnel: w332 -> [w455 w471]
        tunnel: [w450 w466] -> w316
        tunnel: [w447 w463] -> w315
        tunnel: [w446 w462] -> w314
        tunnel: [w445 w461] -> w311
        tunnel: [w444 w460] -> w310
        tunnel: w236 -> [w443 w459]
        tunnel: w236 -> [w442 w458]
        frame True {
          w451 = "BB0131a-R04" ("Changed Product")
          w452 = "90NJ00999" ("SN")
          n110 = call "LabVIEW.Service.Connect_SNDB_with_API_by_HTTPs_Client.vi"("SN"=w452, "Old Product"="BB0131a-R05", "Changed Product"=w451, "error in (no error)"=w455, "Command"=LabVIEW.HTTPs_Client.Command."Vorgang: Migrate serial numbers to a product revision", "Chose Server"=w443) -> ("Result_Cluster"=w446:T4, "Successful?"=w448:bool, "error out"=w454:errorcluster)  [unwired: 11 in, 8 out]
          n111 = call "LabVIEW.Service.Connect_SNDB_with_API_by_HTTPs_Client.vi"("SN"=w452, "Old Product"=w451, "error in (no error)"=w454, "Command"=LabVIEW.HTTPs_Client.Command."Search: Get Seriennummern by Vorgang and Produkt", "Chose Server"=w442) -> ("Result_Cluster"=w444:T4, "Successful?"=w445:bool, "Test other steps"=w449:bool, "error out"=w450:errorcluster)  [unwired: 12 in, 7 out]
          n112 = And(x=w449, y=w448) -> (x .and. y?=w447:bool)
        }
        frame False {
          w467 = "BB0131a-R05" ("Changed Product")
          w468 = "90NJ00999" ("SN")
          n113 = call "LabVIEW.Service.Connect_SNDB_with_API_by_HTTPs_Client.vi"("SN"=w468, "Old Product"="BB0131a-R04", "Changed Product"=w467, "error in (no error)"=w471, "Command"=LabVIEW.HTTPs_Client.Command."Vorgang: Migrate serial numbers to a product revision", "Chose Server"=w459) -> ("Result_Cluster"=w462:T4, "Successful?"=w464:bool, "error out"=w470:errorcluster)  [unwired: 11 in, 8 out]
          n114 = call "LabVIEW.Service.Connect_SNDB_with_API_by_HTTPs_Client.vi"("SN"=w468, "Old Product"=w467, "error in (no error)"=w470, "Command"=LabVIEW.HTTPs_Client.Command."Search: Get Seriennummern by Vorgang and Produkt", "Chose Server"=w458) -> ("Result_Cluster"=w460:T4, "Successful?"=w461:bool, "Test other steps"=w465:bool, "error out"=w466:errorcluster)  [unwired: 12 in, 7 out]
          n115 = And(x=w465, y=w464) -> (x .and. y?=w463:bool)
        }
      }
      n116 = call "LabVIEW.FGV.Creat_Result.vi"("Command"=enum16{"write", "read", "clear"}."write", "error in (no error)"=w316, "Passed?"=w315, "Result_Cluster"=w314) -> ("error out"=w312:errorcluster)  [unwired: 6 in, 1 out]
      n117 = call "LabVIEW.FGV.Creat_Result.vi"("Command"=enum16{"write", "read", "clear"}."write", "error in (no error)"=w312, "Passed?"=w311, "Result_Cluster"=w310) -> ("error out"=w250:errorcluster)  [unwired: 6 in, 1 out]
      n118 = call "LabVIEW.Service.Connect_SNDB_with_API_by_HTTPs_Client.vi"("error in (no error)"=w250, "Command"=LabVIEW.HTTPs_Client.Command."Vorgang: Create test reports(Prüfprotokoll)", "Chose Server"=w236) -> ("Result_Cluster"=w306:T4, "Successful?"=w336:bool, "error out"=w335:errorcluster)  [unwired: 14 in, 8 out]
      n119 = call "LabVIEW.Service.Connect_SNDB_with_API_by_HTTPs_Client.vi"("error in (no error)"=w335, "Command"=LabVIEW.HTTPs_Client.Command."Vorgang: Get serial number data and steps", "Chose Server"=w236) -> ("Body"=w338:string, "error out"=w251:errorcluster)  [unwired: 14 in, 9 out]
      n120 = call "LabVIEW.Service.Connect_SNDB_with_API_by_HTTPs_Client.vi"("error in (no error)"=w251, "Command"=LabVIEW.HTTPs_Client.Command."Seriennummer: Get the text report(Prüfbericht)", "Chose Server"=w236) -> ("Test other steps"=w252:bool, "error out"=w254:errorcluster)  [unwired: 14 in, 9 out]
      n121 = And(x=w252, y=w336) -> (x .and. y?=w307:bool)
      n122 = call "LabVIEW.FGV.Creat_Result.vi"("Command"=enum16{"write", "read", "clear"}."write", "error in (no error)"=w254, "Passed?"=w307, "Result_Cluster"=w306) -> ("error out"=w308:errorcluster)  [unwired: 6 in, 1 out]
      n123 = call <vilib>:"Find Multiple Items.vi"("$Path or Item Name"="$.seriennummern[*].reports[*].fileName", "error in (no error)"=w308, "JSON"=w338) -> ("error out"=w339:errorcluster, "<JSON>"=w340:string[])  [unwired: 5 in, 2 out]
      n124 = for {
        tunnel: w340 -> [w428] mode=indexing
        shift-right: [w425] -> w279
        shift-left: w339 -> [w431]
        tunnel: w236 -> [w424]
        w426 = "90NJ00999" ("Regulärer Ausdruck")
        n125 = call "LabVIEW.FGV.Store_ID.vi"("Command"=enum16{"clear", "write", "read"}."write", "error in (no error)"=w431, "File Name In"=w428) -> ("error out"=w430:errorcluster)  [unwired: 7 in, 5 out]
        n126 = Match Pattern(string=w428, regular expression=w426) -> (offset past match=w429:i32)  [unwired: 1 in, 3 out]
        n127 = Greater Than 0?(x=w429) -> (x > 0?=w427:bool)
        n128 = case shown="False" w427 {
          tunnel: w430 -> [w436 w440]
          tunnel: w426 -> [w435 _]
          tunnel: [w434 w439] -> w425
          tunnel: w424 -> [w433 w438]
          frame True {
            n129 = call "LabVIEW.Service.Connect_SNDB_with_API_by_HTTPs_Client.vi"("SN"=w435, "error in (no error)"=w436, "Command"=LabVIEW.HTTPs_Client.Command."Seriennummer: Delete the text report(Prüfbericht)", "Chose Server"=w433) -> ("error out"=w434:errorcluster)  [unwired: 13 in, 10 out]
          }
          frame False {
            n130 = call "LabVIEW.Service.Connect_SNDB_with_API_by_HTTPs_Client.vi"("error in (no error)"=w440, "Command"=LabVIEW.HTTPs_Client.Command."Seriennummer: Delete the text report(Prüfbericht)", "Chose Server"=w438) -> ("error out"=w439:errorcluster)  [unwired: 14 in, 10 out]
          }
        }
      }
      n131 = disable-structure shown="Disabled" {
        disable-tunnel: w279 -> [w410 w423]
        disable-tunnel: [w402 w423] -> w278
        disable-tunnel: w236 -> [w399 _]
        frame Disabled {
          n132 = call "LabVIEW.HTTPs_Client.Handle_File.vi"("Command"=T3."clear csv", "Fehler (Eingang, kein Fehler)"=w410, "File name"="Test.csv") -> ("Fehler (Ausgang)"=w413:errorcluster, "Successful?"=w415:bool)  [unwired: 7 in]
          n133 = call "LabVIEW.Service.Connect_SNDB_with_API_by_HTTPs_Client.vi"("error in (no error)"=w413, "Command"=LabVIEW.HTTPs_Client.Command."Vorgang: Generate a CSV file", "Chose Server"=w399) -> ("Result_Cluster"=w405:T4, "Successful?"=w416:bool, "error out"=w408:errorcluster)  [unwired: 14 in, 8 out]
          n134 = And(x=w416, y=w415) -> (x .and. y?=w406:bool)
          n135 = call "LabVIEW.FGV.Creat_Result.vi"("Command"=enum16{"write", "read", "clear"}."write", "error in (no error)"=w408, "Passed?"=w406, "Result_Cluster"=w405) -> ("error out"=w407:errorcluster)  [unwired: 6 in, 1 out]
          n136 = call "LabVIEW.HTTPs_Client.Handle_File.vi"("Command"=T3."clear xlsx", "Fehler (Eingang, kein Fehler)"=w407, "File name"="Test.xlsx") -> ("Fehler (Ausgang)"=w420:errorcluster, "Successful?"=w421:bool)  [unwired: 7 in]
          n137 = call "LabVIEW.Service.Connect_SNDB_with_API_by_HTTPs_Client.vi"("error in (no error)"=w420, "Command"=LabVIEW.HTTPs_Client.Command."Vorgang: Generate an XLSX file", "Chose Server"=w399) -> ("Result_Cluster"=w400:T4, "Successful?"=w422:bool, "error out"=w403:errorcluster)  [unwired: 14 in, 8 out]
          n138 = And(x=w422, y=w421) -> (x .and. y?=w401:bool)
          n139 = call "LabVIEW.FGV.Creat_Result.vi"("Command"=enum16{"write", "read", "clear"}."write", "error in (no error)"=w403, "Passed?"=w401, "Result_Cluster"=w400) -> ("error out"=w402:errorcluster)  [unwired: 6 in, 1 out]
        }
        frame Enabled {
        }
      }
      n140 = call "LabVIEW.Service.Connect_SNDB_with_API_by_HTTPs_Client.vi"("error in (no error)"=w278, "Command"=LabVIEW.HTTPs_Client.Command."Fertigmeldung: Create a Fertigmeldung", "Chose Server"=w236) -> ("Result_Cluster"=w274:T4, "Successful?"=w291:bool, "error out"=w287:errorcluster)  [unwired: 14 in, 8 out]
      n141 = call "LabVIEW.Service.Connect_SNDB_with_API_by_HTTPs_Client.vi"("error in (no error)"=w287, "Command"=LabVIEW.HTTPs_Client.Command."Vorgang: Get serial number data and steps", "Chose Server"=w236) -> ("error out"=w288:errorcluster)  [unwired: 14 in, 10 out]
      n142 = call "LabVIEW.FGV.Store_ID.vi"("Command"=enum16{"clear", "write", "read"}."read", "error in (no error)"=w288) -> ("Fertigmeldung out[]"=w282:string[], "error out"=w286:errorcluster)  [unwired: 8 in, 4 out]
      n143 = Index Array(array=w282, index=0 ("Index")) -> (element=w284:string)
      n144 = Equal?(x=w284, y="true") -> (x = y?=w290:bool)
      n145 = call "LabVIEW.Service.Connect_SNDB_with_API_by_HTTPs_Client.vi"("error in (no error)"=w286, "Command"=LabVIEW.HTTPs_Client.Command."Vorgang: Get a CSV file(Fertigmeldung report)", "Chose Server"=w236) -> ("Result_Cluster"=w269:T4, "Successful?"=w270:bool, "error out"=w276:errorcluster)  [unwired: 14 in, 8 out]
      n146 = Compound Arithmetic op=AND ("Mehrfacharithmetik")(w270, w290, w291) -> (w275:bool)
      n147 = call "LabVIEW.FGV.Creat_Result.vi"("Command"=enum16{"write", "read", "clear"}."write", "error in (no error)"=w276, "Passed?"=w275, "Result_Cluster"=w274) -> ("error out"=w272:errorcluster)  [unwired: 6 in, 1 out]
      n148 = call "LabVIEW.FGV.Creat_Result.vi"("Command"=enum16{"write", "read", "clear"}."write", "error in (no error)"=w272, "Passed?"=w270, "Result_Cluster"=w269) -> ("error out"=w271:errorcluster)  [unwired: 6 in, 1 out]
      n149 = call "LabVIEW.Service.Connect_SNDB_with_API_by_HTTPs_Client.vi"("error in (no error)"=w271, "Command"=LabVIEW.HTTPs_Client.Command."Fertigmeldung: Revert the Fertigmeldung", "Chose Server"=w236) -> ("Result_Cluster"=w264:T4, "Successful?"=w301:bool, "error out"=w296:errorcluster)  [unwired: 14 in, 8 out]
      n150 = call "LabVIEW.Service.Connect_SNDB_with_API_by_HTTPs_Client.vi"("error in (no error)"=w296, "Command"=LabVIEW.HTTPs_Client.Command."Vorgang: Get serial number data and steps", "Chose Server"=w236) -> ("error out"=w294:errorcluster)  [unwired: 14 in, 10 out]
      n151 = call "LabVIEW.FGV.Store_ID.vi"("Command"=enum16{"clear", "write", "read"}."read", "error in (no error)"=w294) -> ("Fertigmeldung out[]"=w293:string[], "error out"=w267:errorcluster)  [unwired: 8 in, 4 out]
      n152 = Index Array(array=w293, index=0 ("Index")) -> (element=w297:string)
      n153 = Equal?(x=w297, y="false") -> (x = y?=w300:bool)
      n154 = And(x=w300, y=w301) -> (x .and. y?=w265:bool)
      n155 = call "LabVIEW.FGV.Creat_Result.vi"("Command"=enum16{"write", "read", "clear"}."write", "error in (no error)"=w267, "Passed?"=w265, "Result_Cluster"=w264) -> ("error out"=w266:errorcluster)  [unwired: 6 in, 1 out]
      n156 = call "LabVIEW.Service.Connect_SNDB_with_API_by_HTTPs_Client.vi"("error in (no error)"=w266, "Command"=LabVIEW.HTTPs_Client.Command."Search: Get Vorgang/Produkt combinations", "Chose Server"=w236) -> ("Result_Cluster"=w261:T4, "Successful?"=w260:bool, "error out"=w262:errorcluster)  [unwired: 14 in, 8 out]
      n157 = call "LabVIEW.FGV.Creat_Result.vi"("Command"=enum16{"write", "read", "clear"}."write", "error in (no error)"=w262, "Passed?"=w260, "Result_Cluster"=w261) -> ("error out"=w259:errorcluster)  [unwired: 6 in, 1 out]
      n158 = call "LabVIEW.Service.Connect_SNDB_with_API_by_HTTPs_Client.vi"("error in (no error)"=w259, "Command"=LabVIEW.HTTPs_Client.Command."Search: Lookup Vorgang", "Chose Server"=w236) -> ("Result_Cluster"=w256:T4, "Successful?"=w255:bool, "error out"=w257:errorcluster)  [unwired: 14 in, 8 out]
      n159 = call "LabVIEW.FGV.Creat_Result.vi"("Command"=enum16{"write", "read", "clear"}."write", "error in (no error)"=w257, "Passed?"=w255, "Result_Cluster"=w256) -> ("error out"=w244:errorcluster)  [unwired: 6 in, 1 out]
      n160 = call "LabVIEW.Service.Connect_SNDB_with_API_by_HTTPs_Client.vi"("error in (no error)"=w244, "Command"=LabVIEW.HTTPs_Client.Command."Search: Find production plan", "Chose Server"=w236) -> ("Result_Cluster"=w248:T4, "Successful?"=w249:bool, "error out"=w247:errorcluster)  [unwired: 14 in, 8 out]
      n161 = call "LabVIEW.FGV.Creat_Result.vi"("Command"=enum16{"write", "read", "clear"}."write", "error in (no error)"=w247, "Passed?"=w249, "Result_Cluster"=w248) -> ("error out"=w238:errorcluster)  [unwired: 6 in, 1 out]
      n162 = call "LabVIEW.Service.Connect_SNDB_with_API_by_HTTPs_Client.vi"("error in (no error)"=w238, "Command"=LabVIEW.HTTPs_Client.Command."Search: Find production plan arrangement", "Chose Server"=w236) -> ("Result_Cluster"=w240:T4, "Successful?"=w239:bool, "error out"=w241:errorcluster)  [unwired: 14 in, 8 out]
      n163 = call "LabVIEW.FGV.Creat_Result.vi"("Command"=enum16{"write", "read", "clear"}."write", "error in (no error)"=w241, "Passed?"=w239, "Result_Cluster"=w240) -> ("error out"=w237:errorcluster)  [unwired: 6 in, 1 out]
    }
    frame "Test User/Role/Permission" {
      n164 = call "LabVIEW.Service.Connect_SNDB_with_API_by_HTTPs_Client.vi"("error in (no error)"=w531, "Command"=LabVIEW.HTTPs_Client.Command."User: Get all users", "Chose Server"=w502) -> ("Result_Cluster"=w527:T4, "Successful?"=w526:bool, "Body"=w542:string, "error out"=w529:errorcluster)  [unwired: 14 in, 7 out]
      n165 = call "LabVIEW.FGV.Creat_Result.vi"("Command"=enum16{"write", "read", "clear"}."write", "error in (no error)"=w529, "Passed?"=w526, "Result_Cluster"=w527) -> ("error out"=w528:errorcluster)  [unwired: 6 in, 1 out]
      n166 = call <vilib>:"Find Multiple Items.vi"("$Path or Item Name"="$[*].username", "error in (no error)"=w528, "JSON"=w542) -> ("error out"=w537:errorcluster, "<JSON>"=w535:string[])  [unwired: 5 in, 2 out]
      n167 = Search 1D Array(1D array=w535, element="\"test\"" ("Element")) -> (index of element=w539:i32)  [unwired: 1 in]
      n168 = call <vilib>:"Find Multiple Items.vi"("$Path or Item Name"="$[*].infoText", "error in (no error)"=w537, "JSON"=w542) -> ("error out"=w544:errorcluster, "<JSON>"=w538:string[])  [unwired: 5 in, 2 out]
      n169 = Index Array(array=w538, index=w539) -> (element=w540:string)
      n170 = Equal?(x=w540, y="\"\"" ("Info text")) -> (x = y?=w545:bool)
      n171 = call "LabVIEW.Service.Connect_SNDB_with_API_by_HTTPs_Client.vi"("error in (no error)"=w544, "Command"=LabVIEW.HTTPs_Client.Command."User: Get all user roles", "Chose Server"=w502) -> ("Result_Cluster"=w522:T4, "Successful?"=w521:bool, "error out"=w524:errorcluster)  [unwired: 14 in, 8 out]
      n172 = call "LabVIEW.FGV.Creat_Result.vi"("Command"=enum16{"write", "read", "clear"}."write", "error in (no error)"=w524, "Passed?"=w521, "Result_Cluster"=w522) -> ("error out"=w523:errorcluster)  [unwired: 6 in, 1 out]
      n173 = case shown="True" w545 {
        tunnel: [w566 w580] -> w547
        tunnel: [w565 w579] -> w546
        tunnel: w523 -> [w564 w578]
        tunnel: [w562 w575] -> w519
        tunnel: [w561 w574] -> w512
        tunnel: [w560 w573] -> w517
        tunnel: [w559 w572] -> w513
        tunnel: w502 -> [w558 w571]
        tunnel: w502 -> [w557 w570]
        frame True {
          w563 = "\"Test_infoText\"" ("Info text")
          n174 = call "LabVIEW.Service.Connect_SNDB_with_API_by_HTTPs_Client.vi"("error in (no error)"=w564, "Command"=LabVIEW.HTTPs_Client.Command."User: Update an user", "Info text"=w563, "Chose Server"=w558) -> ("Result_Cluster"=w560:T4, "Successful?"=w566:bool, "error out"=w567:errorcluster)  [unwired: 13 in, 8 out]
          n175 = call "LabVIEW.Service.Connect_SNDB_with_API_by_HTTPs_Client.vi"("error in (no error)"=w567, "Command"=LabVIEW.HTTPs_Client.Command."User: Get a single user", "Info text"=w563, "Chose Server"=w557) -> ("Result_Cluster"=w559:T4, "Successful?"=w561:bool, "Test other steps"=w565:bool, "error out"=w562:errorcluster)  [unwired: 13 in, 7 out]
        }
        frame False {
          n176 = call "LabVIEW.Service.Connect_SNDB_with_API_by_HTTPs_Client.vi"("error in (no error)"=w578, "Command"=LabVIEW.HTTPs_Client.Command."User: Update an user", "Info text"="null", "Chose Server"=w571) -> ("Result_Cluster"=w573:T4, "Successful?"=w580:bool, "error out"=w581:errorcluster)  [unwired: 13 in, 8 out]
          n177 = call "LabVIEW.Service.Connect_SNDB_with_API_by_HTTPs_Client.vi"("error in (no error)"=w581, "Command"=LabVIEW.HTTPs_Client.Command."User: Get a single user", "Info text"="\"\"", "Chose Server"=w570) -> ("Result_Cluster"=w572:T4, "Successful?"=w574:bool, "Test other steps"=w579:bool, "error out"=w575:errorcluster)  [unwired: 13 in, 7 out]
        }
      }
      n178 = And(x=w546, y=w547) -> (x .and. y?=w518:bool)
      n179 = call "LabVIEW.FGV.Creat_Result.vi"("Command"=enum16{"write", "read", "clear"}."write", "error in (no error)"=w519, "Passed?"=w518, "Result_Cluster"=w517) -> ("error out"=w515:errorcluster)  [unwired: 6 in, 1 out]
      n180 = call "LabVIEW.FGV.Creat_Result.vi"("Command"=enum16{"write", "read", "clear"}."write", "error in (no error)"=w515, "Passed?"=w512, "Result_Cluster"=w513) -> ("error out"=w514:errorcluster)  [unwired: 6 in, 1 out]
      n181 = call "LabVIEW.Service.Connect_SNDB_with_API_by_HTTPs_Client.vi"("error in (no error)"=w514, "Command"=LabVIEW.HTTPs_Client.Command."User: Get a single user role", "Chose Server"=w502) -> ("Result_Cluster"=w508:T4, "Successful?"=w507:bool, "Body"=w553:string, "error out"=w510:errorcluster)  [unwired: 14 in, 7 out]
      n182 = call "LabVIEW.FGV.Creat_Result.vi"("Command"=enum16{"write", "read", "clear"}."write", "error in (no error)"=w510, "Passed?"=w507, "Result_Cluster"=w508) -> ("error out"=w509:errorcluster)  [unwired: 6 in, 1 out]
      n183 = call <vilib>:"Find Multiple Items.vi"("$Path or Item Name"="$.permissions[*]", "error in (no error)"=w509, "JSON"=w553) -> ("error out"=w501:errorcluster, "<JSON>"=w550:string[])  [unwired: 5 in, 2 out]
      n184 = Search 1D Array(1D array=w550, element="\"sn_run_dispach_step\"" ("Neues Element/Teil-Array")) -> (index of element=w552:i32)  [unwired: 1 in]
      n185 = Greater Or Equal To 0?(x=w552) -> (x >= 0?=w554:bool)
      n186 = Not(x=w554) -> (.not. x?=w556:bool)
      n187 = call "LabVIEW.Service.Connect_SNDB_with_API_by_HTTPs_Client.vi"("error in (no error)"=w501, "Command"=LabVIEW.HTTPs_Client.Command."User: Get all permissions", "Chose Server"=w502, "User Update user role\"sn_run_dispach_step\""=w556) -> ("Result_Cluster"=w504:T4, "Successful?"=w505:bool, "error out"=w500:errorcluster)  [unwired: 13 in, 8 out]
      n188 = call "LabVIEW.FGV.Creat_Result.vi"("Command"=enum16{"write", "read", "clear"}."write", "error in (no error)"=w500, "Passed?"=w505, "Result_Cluster"=w504) -> ("error out"=w503:errorcluster)  [unwired: 6 in, 1 out]
    }
    frame "Test MAC addresses" {
      n189 = call "LabVIEW.Service.Connect_SNDB_with_API_by_HTTPs_Client.vi"("error in (no error)"=w600, "Command"=LabVIEW.HTTPs_Client.Command."MAC addresses: Get all reserved MAC addresses", "Chose Server"=w584) -> ("Result_Cluster"=w596:T4, "Successful?"=w595:bool, "error out"=w598:errorcluster)  [unwired: 14 in, 8 out]
      n190 = call "LabVIEW.FGV.Creat_Result.vi"("Command"=enum16{"write", "read", "clear"}."write", "error in (no error)"=w598, "Passed?"=w595, "Result_Cluster"=w596) -> ("error out"=w597:errorcluster)  [unwired: 6 in, 1 out]
      n191 = call "LabVIEW.Service.Connect_SNDB_with_API_by_HTTPs_Client.vi"("error in (no error)"=w597, "Command"=LabVIEW.HTTPs_Client.Command."MAC addresses: Get the most recently reserved MAC addresses", "Chose Server"=w584) -> ("Result_Cluster"=w591:T4, "Successful?"=w590:bool, "error out"=w593:errorcluster)  [unwired: 14 in, 8 out]
      n192 = call "LabVIEW.FGV.Creat_Result.vi"("Command"=enum16{"write", "read", "clear"}."write", "error in (no error)"=w593, "Passed?"=w590, "Result_Cluster"=w591) -> ("error out"=w592:errorcluster)  [unwired: 6 in, 1 out]
      n193 = call "LabVIEW.Service.Connect_SNDB_with_API_by_HTTPs_Client.vi"("error in (no error)"=w592, "Command"=LabVIEW.HTTPs_Client.Command."MAC addresses: Get data for a MAC address", "Chose Server"=w584) -> ("Result_Cluster"=w586:T4, "Successful?"=w585:bool, "error out"=w588:errorcluster)  [unwired: 14 in, 8 out]
      n194 = call "LabVIEW.FGV.Creat_Result.vi"("Command"=enum16{"write", "read", "clear"}."write", "error in (no error)"=w588, "Passed?"=w585, "Result_Cluster"=w586) -> ("error out"=w587:errorcluster)  [unwired: 6 in, 1 out]
    }
    frame "Test Health check" {
      n195 = call "LabVIEW.Service.Connect_SNDB_with_API_by_HTTPs_Client.vi"("error in (no error)"=w605, "Command"=LabVIEW.HTTPs_Client.Command."Health check: Health check", "Chose Server"=w606) -> ("Result_Cluster"=w608:T4, "Successful?"=w607:bool, "error out"=w609:errorcluster)  [unwired: 14 in, 8 out]
      n196 = call "LabVIEW.FGV.Creat_Result.vi"("Command"=enum16{"write", "read", "clear"}."write", "error in (no error)"=w609, "Passed?"=w607, "Result_Cluster"=w608) -> ("error out"=w604:errorcluster)  [unwired: 6 in, 1 out]
    }
    frame " Test Authentication at the end" {
      n197 = call "LabVIEW.Service.Connect_SNDB_with_API_by_HTTPs_Client.vi"("error in (no error)"=w617, "Command"=LabVIEW.HTTPs_Client.Command."Authentication: Revoke the token", "Chose Server"=w612) -> ("Result_Cluster"=w614:T4, "Successful?"=w613:bool, "error out"=w616:errorcluster)  [unwired: 14 in, 8 out]
      n198 = call "LabVIEW.FGV.Creat_Result.vi"("Command"=enum16{"write", "read", "clear"}."write", "error in (no error)"=w616, "Passed?"=w613, "Result_Cluster"=w614) -> ("error out"=w615:errorcluster)  [unwired: 6 in, 1 out]
    }
  }
  "Fehler (Ausgang)" <- w3
